vi "GetRightClickMenu.vi"(0 "reference":refnum<class "ClassDiagramGraph.lvclass">, 5 "error in (no error)":errorcluster) -> (14 "reference out":refnum<class "ClassDiagramGraph.lvclass">, 15 "Array":string[](array[string]), 16 "Found":bool, 19 "error out":errorcluster)   [LabVIEW 2020, in "ClassDiagramGraph.lvclass"]
uses:
  <resource>/Framework/Providers/Open_GDS/UML/ClassDiagramGraph_class/ClassDiagramGraph.lvclass
  C:/Program Files (x86)/National Instruments/LabVIEW 2020/resource/Framework/Providers/Open_GDS/UML/Graph_class/Graph.lvclass
  <resource>/Framework/Providers/Open_GDS/UML/ClassNode_class/ClassNode.lvclass
  C:/Program Files (x86)/National Instruments/LabVIEW 2020/resource/Framework/Providers/Open_GDS/UML/AbstractNode_class/AbstractNode.lvclass
  <resource>/Framework/Providers/Open_GDS/UML/AbstractNode_class/AbstractNode.lvclass
  <resource>/Framework/Providers/Open_GDS/UML/Graph_class/Graph.lvclass
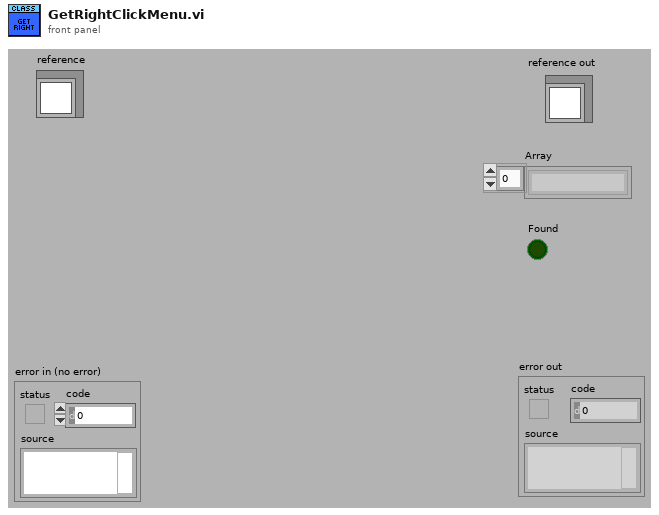
[diagram p1: front panel]
types:
  T1 = typedef "Graph.lvclass/ObjectAttributes.ctl" = cluster{"nodes":refnum<class "AbstractNode.lvclass">[], "edges":refnum<class "AbstractEdge.lvclass">[], "nodesToBeRemoved":refnum<class "AbstractNode.lvclass">[], "edgesToBeRemoved":refnum<class "AbstractEdge.lvclass">[], "needsLayout":bool, "LayoutNodes":refnum<class "AbstractNode.lvclass">[]}
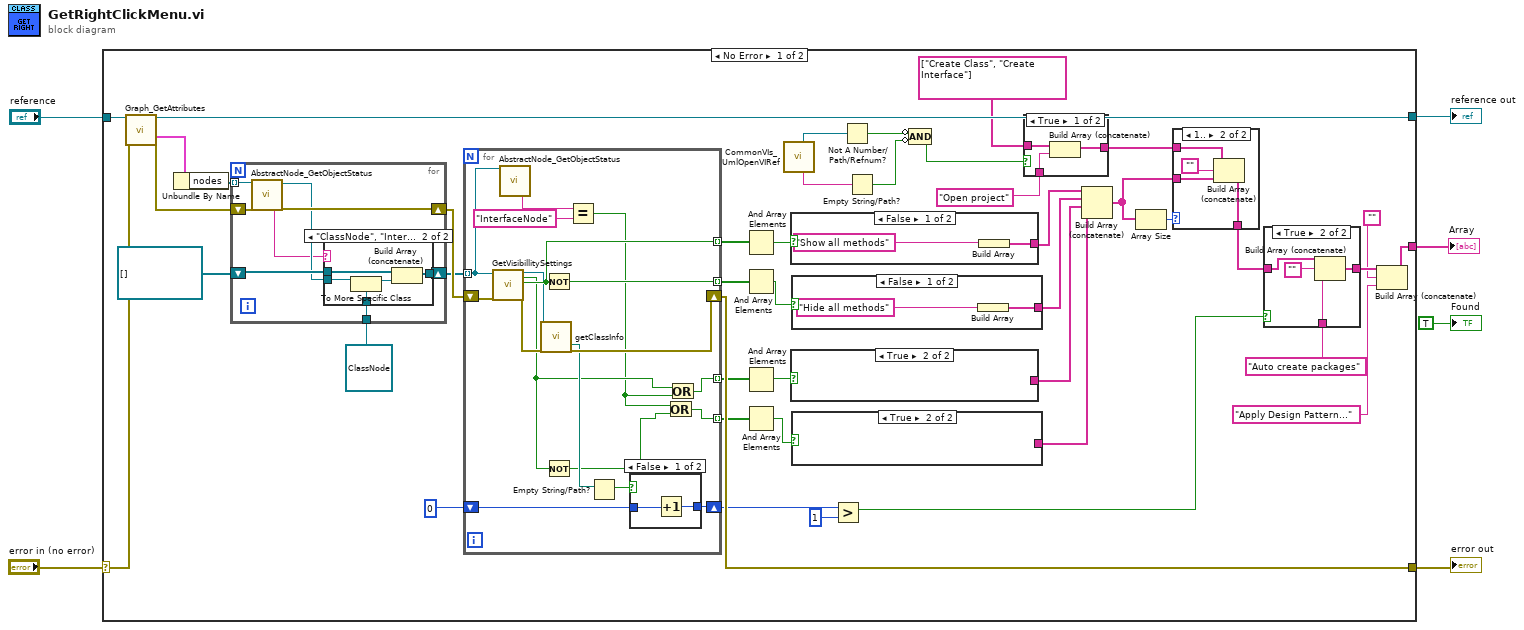
[diagram p0: block diagram]
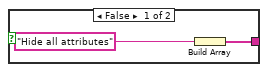
[diagram p4: hidden frame]
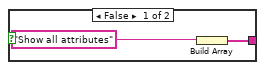
[diagram p5: hidden frame]
diagram:
  n1 = case shown="No Error" "error in (no error)" {
    selector: "error in (no error)" -> [w49 w107]
    tunnel: "reference" -> [w48 w108]
    tunnel: [w43 w107] -> w4
    tunnel: [w47 w108] -> w3
    tunnel: [w10 _] -> w2
    frame No Error {
      n2 = call <resource>:"Graph_GetAttributes.vi"("reference in"=w48, "error in (no error)"=w49) -> ("reference out"=w47:refnum<class "ClassDiagramGraph.lvclass">, "Data"=w7:T1, "error out"=w44:errorcluster)  [unwired: 14 in, 1 out]
      n3 = Unbundle By Name(w7) -> ("nodes"=w19:refnum<class "AbstractNode.lvclass">[])
      n4 = for {
        shift-right: [w98] -> w45
        shift-left: w44 -> [w100]
        tunnel: w19 -> [w99] mode=indexing
        shift-right: [w95] -> w17
        shift-left: refnum<class "ClassNode.lvclass">[] [] -> [w97]
        tunnel: refnum<class "ClassNode.lvclass"> refnum ("reference out") -> [w94]
        n5 = call <resource>:"AbstractNode_GetObjectStatus.vi"("reference in"=w99, "error in (no error)"=w100) -> ("Class name"=w93:string, "reference out"=w96:refnum<class "AbstractNode.lvclass">, "error out"=w98:errorcluster)  [unwired: 15 out]
        n6 = case shown="\"ClassNode\", \"InterfaceNode\"" w93 {
          tunnel: w97 -> [w101 w106]
          tunnel: w96 -> [_ w104]
          tunnel: [w101 w105] -> w95
          tunnel: w94 -> [_ w102]
          frame Default {
          }
          frame "ClassNode", "InterfaceNode" {
            n7 = To More Specific Class(target class=w102, reference=w104) -> (specific class reference=w103:refnum<class "ClassNode.lvclass">)  [unwired: 1 in, 1 out]
            n8 = Build Array (concatenate)(w106, w103) -> (w105:refnum<class "ClassNode.lvclass">[])
          }
        }
      }
      n9 = for {
        tunnel: w17 -> [w79] mode=indexing
        shift-right: [w85] -> w43
        shift-left: w45 -> [w89]
        tunnel: [w88] -> w39 mode=indexing
        tunnel: [w87] -> w40 mode=indexing
        tunnel: [w72] -> w34 mode=indexing
        tunnel: [w77] -> w33 mode=indexing
        shift-right: [w80] -> w15
        shift-left: 0 ("y") -> [w81]
        n10 = call <resource>:"GetVisibillitySettings.vi"("reference"=w79, "error in (no error)"=w89) -> ("reference out"=w83:refnum<class "ClassNode.lvclass">, "showAttribute"=w78:bool, "showMethods"=w87:bool, "error out"=w86:errorcluster)  [unwired: 14 out]
        n11 = call <resource>:"AbstractNode_GetObjectStatus.vi"("reference in"=w79) -> ("Class name"=w75:string)  [unwired: 1 in, 17 out]
        n12 = call-dynamic "getClassInfo.vi"("reference"=w83, "error in (no error)"=w86) -> ("ClassPath"=w84:path, "error out"=w85:errorcluster)  [unwired: 8 in, 8 out]
        n13 = Not(x=w87) -> (.not. x?=w88:bool)
        n14 = Not(x=w78) -> (.not. x?=w76:bool)
        n15 = Equal?(x=w75, y="InterfaceNode") -> (x = y?=w73:bool)
        n16 = Empty String/Path?(string/path=w84) -> (empty?=w82:bool)
        n17 = case shown="False" w82 {
          tunnel: w81 -> [w91 w92]
          tunnel: [w90 w92] -> w80
          frame False {
            n18 = Increment(x=w91) -> (x+1=w90:i32)
          }
          frame True {
          }
        }
        n19 = Or(x=w73, y=w76) -> (x .or. y?=w72:bool)
        n20 = Or(x=w78, y=w73) -> (x .or. y?=w77:bool)
      }
      n21 = And Array Elements(Boolean array=w40) -> (logical AND=w38:bool)
      n22 = And Array Elements(Boolean array=w39) -> (logical AND=w37:bool)
      n23 = And Array Elements(Boolean array=w33) -> (logical AND=w32:bool)
      n24 = And Array Elements(Boolean array=w34) -> (logical AND=w31:bool)
      n25 = call <resource>:"CommonVIs_UmlOpenVIRef.vi"() -> ("ProjectNameOut"=w25:string, "AppRefOut"=w26:refnum<vi>)  [unwired: 4 in, 6 out]
      n26 = case shown="False" w38 {
        tunnel: [w71 _] -> w42
        frame False {
          n27 = Build Array("Show all methods") -> (w71:string[])
        }
        frame True {
        }
      }
      n28 = case shown="True" w32 {
        tunnel: [w62 _] -> w30
        frame False {
          n29 = Build Array("Show all attributes") -> (w62:string[])
        }
        frame True {
        }
      }
      n30 = case shown="False" w37 {
        tunnel: [w69 _] -> w41
        frame False {
          n31 = Build Array("Hide all methods") -> (w69:string[])
        }
        frame True {
        }
      }
      n32 = case shown="True" w31 {
        tunnel: [w60 _] -> w29
        frame False {
          n33 = Build Array("Hide all attributes") -> (w60:string[])
        }
        frame True {
        }
      }
      n34 = Greater?(x=w15, y=1) -> (0:w13:bool)
      n35 = Not A Number/Path/Refnum?(number/path/refnum=w26) -> (NaN/Path/Refnum?=w24:bool)
      n36 = Empty String/Path?(string/path=w25) -> (empty?=w23:bool)
      n37 = Compound Arithmetic op=AND(invert w24, invert w23) -> (w22:bool)
      n38 = case shown="True" w22 {
        tunnel: string[] ["Create Class", "Create Interface"] -> [w57 w58]
        tunnel: [w56 w58] -> w27
        tunnel: "Open project" ("element") -> [w55 _]
        frame True {
          n39 = Build Array (concatenate)(w57, w55) -> (w56:string[])
        }
        frame False {
        }
      }
      n40 = Build Array (concatenate)(w42, w41, w30, w29) -> (w36:string[])
      n41 = Array Size(array=w36) -> (size(s)=w35:i32)
      n42 = case shown="1.." w35 {
        tunnel: [w63 w67] -> w14
        tunnel: w27 -> [w63 w66]
        tunnel: w36 -> [_ w65]
        frame Default {
        }
        frame 1.. {
          n43 = Build Array (concatenate)(w66, "", w65) -> (w67:string[])
        }
      }
      n44 = case shown="True" w13 {
        tunnel: w14 -> [w50 w52]
        tunnel: [w50 w53] -> w11
        tunnel: "Auto create packages" -> [_ w51]
        frame False {
        }
        frame True {
          n45 = Build Array (concatenate)(w52, "", w51) -> (w53:string[])
        }
      }
      n46 = Build Array (concatenate)(w11, "", "Apply Design Pattern..." ("element")) -> (w10:string[])
    }
    frame Error {
    }
  }
  "reference out" <- w3
  "error out" <- w4
  "Array" <- w2
  "Found" <- TRUE ("Found")
